vi "Workspace Experiment reload.vi"() -> ()   [LabVIEW 2023]
uses:
  <vilib>/Comparison/Equal/Equal Functor/Equal Functor.lvclass
  c59a542d-4e72-4e5b-a943-7cf77955b126.vi
  68731def-adea-4c2f-8935-8a66735695fa.vi
  <vilib>/Utility/sysdir.llb/System Directory Type.ctl
panel:
  out "output cluster":T1
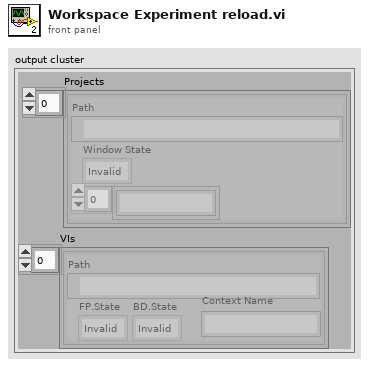
[diagram p1: front panel]
types:
  T1 = cluster{"Projects":cluster{"Path":path, "Window State":enum32{"Invalid", "Standard", "Closed", "Hidden", "Minimized", "Maximized"}, string[]}[], "VIs":cluster{"Path":path, "Context Name":string, "FP.State":enum32{"Invalid", "Standard", "Closed", "Hidden", "Minimized", "Maximized"}, "BD.State":enum32{"Invalid", "Standard", "Closed", "Hidden", "Minimized", "Maximized"}}[]}
  T2 = typedef "System Directory Type.ctl" = i32
  T3 = cluster{"Projects":cluster{"Path":path, "Window State":enum32{"Invalid", "Standard", "Closed", "Hidden", "Minimized", "Maximized"}, string[]}[], "VIs":cluster{"Path":path, string, "FP.State":enum32{"Invalid", "Standard", "Closed", "Hidden", "Minimized", "Maximized"}, "BD.State":enum32{"Invalid", "Standard", "Closed", "Hidden", "Minimized", "Maximized"}}[]}
  T4 = cluster{"Path":path, "Window State":enum32{"Invalid", "Standard", "Closed", "Hidden", "Minimized", "Maximized"}, string[]}[]
  T5 = cluster{"Path":path, string, "FP.State":enum32{"Invalid", "Standard", "Closed", "Hidden", "Minimized", "Maximized"}, "BD.State":enum32{"Invalid", "Standard", "Closed", "Hidden", "Minimized", "Maximized"}}[]
  T6 = enum32{"Invalid", "Standard", "Closed", "Hidden", "Minimized", "Maximized"}
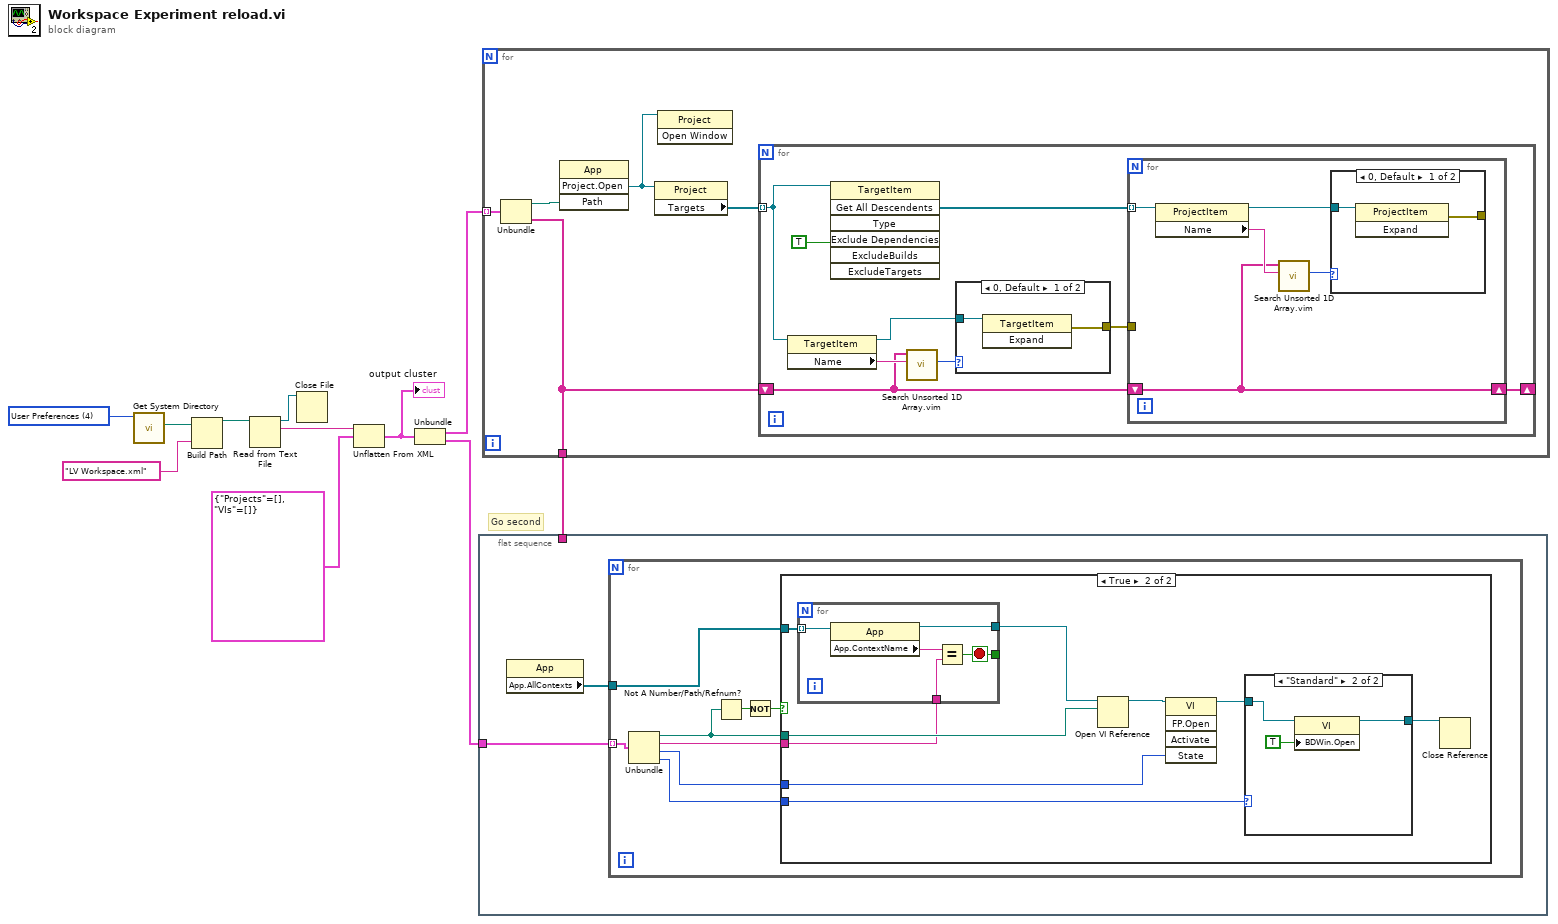
[diagram p0: block diagram]
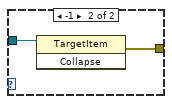
[diagram p4: hidden frame]
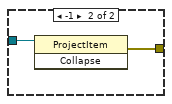
[diagram p5: hidden frame]
diagram:
  w3 = T2 4 items=["User Home"=0, "User Desktop"=1, "User Documents"=2, "User Application Data"=3, "User Preferences"=4, "User Temporary"=5, "Public Documents"=6, "Public Application Data"=7, "Public Preferences"=8, "Public Cache"=13, "System Core Libraries"=9, "System Installed Libraries"=10, "Application Files"=11, "Boot Volume Root"=12] ("system directory type")
  # "Go second"
  n1 = call <vilib>:"Get System Directory.vi"("system directory type"=w3) -> ("system directory"=w4:path)  [unwired: 10 in]
  n2 = Build Path(base path=w4, name or relative path="LV Workspace.xml") -> (appended path=w2:path)
  n3 = Read from Text File(file (use dialog)=w2) -> (refnum out=w6:refnum<file>, text=w7:string)  [unwired: 3 in, 2 out]
  n4 = Close File(refnum=w6) -> ()  [unwired: 1 in, 2 out]
  n5 = Unflatten From XML(xml string=w7, type=T3 {"Projects"=[], "VIs"=[]} ("output cluster")) -> (value=w8:T3)  [unwired: 1 in, 1 out]
  "output cluster" <- w8
  n6 = Unbundle(w8) -> ("Projects"=w10:T4, "VIs"=w11:T5)
  n7 = flat-sequence {
    tunnel: w11 -> [w13]
    tunnel: w1 -> [_]
    frame #0 {
      n8 = property class="App"() -> ("App.AllContexts"=w12:refnum<vi>[])  [unwired: 2 in, 2 out]
      n9 = for {
        tunnel: w13 -> [w21] mode=indexing
        tunnel: w12 -> [w17]
        n10 = Unbundle(w21) -> ("Path"=w18:path, w14:string, "FP.State"=w15:T6, "BD.State"=w16:T6)
        n11 = Not A Number/Path/Refnum?(number/path/refnum=w18) -> (NaN/Path/Refnum?=w20:bool)
        n12 = Not(x=w20) -> (.not. x?=w19:bool)
        n13 = case shown="True" w19 {
          tunnel: w18 -> [_ w30]
          tunnel: w15 -> [_ w28]
          tunnel: w16 -> [_ w27]
          tunnel: w17 -> [_ w24]
          tunnel: w14 -> [_ w23]
          frame False {
          }
          frame True {
            n14 = for {
              tunnel: w24 -> [w31] mode=indexing
              tunnel: w23 -> [w35]
              tunnel: [w32] -> w22
              tunnel: [w33] -> _
              stop <- w33 stop-if-true
              n15 = property class="App"(reference=w31) -> (reference out=w32:refnum<vi>, "App.ContextName"=w34:string)  [unwired: 1 in, 1 out]
              n16 = Equal?(x=w34, y=w35) -> (x = y?=w33:bool)
            }
            n17 = Open VI Reference(application reference (local)=w22, vi path=w30) -> (vi reference=w29:refnum<vi>)  [unwired: 4 in, 1 out]
            n18 = invoke class="VI" method="FP.Open"(reference=w29, "State"=w28) -> (reference out=w26:refnum<vi>)  [unwired: 3 in, 4 out]
            n19 = case shown="\"Standard\"" w27 {
              tunnel: w26 -> [w36 w39]
              tunnel: [w36 w37] -> w25
              frame "Invalid", Default {
              }
              frame "Standard" {
                n20 = property class="VI"(reference=w39, "BDWin.Open"=TRUE ("Block Diagram Window:Open")) -> (reference out=w37:refnum<vi>)  [unwired: 1 in, 1 out]
              }
            }
            n21 = Close Reference(reference=w25) -> ()  [unwired: 1 in, 1 out]
          }
        }
      }
    }
  }
  n22 = for {
    tunnel: w10 -> [w44] mode=indexing
    tunnel: [w41] -> w1
    n23 = Unbundle(w44) -> ("Path"=w43:path, w41:string[])  [unwired: 1 out]
    n24 = invoke class="App" method="Project.Open"("Path"=w43) -> ("Project:Open"=w40:refnum<vi>)  [unwired: 3 in, 3 out]
    n25 = property class="Project"(reference=w40) -> ("Targets"=w42:refnum<vi>[])  [unwired: 1 in, 2 out]
    n26 = invoke class="Project" method="Open Window"(reference=w40) -> ()  [unwired: 2 in, 3 out]
    n27 = for {
      tunnel: w42 -> [w51] mode=indexing
      shift-right: [w52] -> _
      shift-left: w41 -> [w48]
      n28 = property class="TargetItem"(reference=w51) -> (reference out=w46:refnum<vi>, "Name"=w49:string)  [unwired: 1 in, 1 out]
      n29 = invoke class="TargetItem" method="Get All Descendents"(reference=w51, "Exclude Dependencies"=TRUE ("ExcludeDependencies")) -> ("All Descendents"=w53:refnum<vi>[])  [unwired: 5 in, 6 out]
      n30 = call "Search Unsorted 1D Array.vim"("element"=w49, "unsorted 1D array"=w48) -> ("index of element"=w47:i32)  [unwired: 9 in]
      n31 = case shown="0, Default" w47 {
        tunnel: w46 -> [w55 w57]
        tunnel: [w54 w56] -> w45
        frame 0, Default {
          n32 = invoke class="TargetItem" method="Expand"(reference=w55) -> (error out=w54:errorcluster)  [unwired: 2 in, 2 out]
        }
        frame -1 {
          n33 = invoke class="TargetItem" method="Collapse"(reference=w57) -> (error out=w56:errorcluster)  [unwired: 2 in, 2 out]
        }
      }
      n34 = for {
        tunnel: w53 -> [w61] mode=indexing
        shift-right: [w58] -> w52
        shift-left: w48 -> [w58]
        tunnel: w45 -> [_]
        n35 = property class="ProjectItem"(reference=w61) -> (reference out=w62:refnum<vi>, "Name"=w60:string)  [unwired: 1 in, 1 out]
        n36 = call "Search Unsorted 1D Array.vim"("element"=w60, "unsorted 1D array"=w58) -> ("index of element"=w59:i32)  [unwired: 9 in]
        n37 = case shown="0, Default" w59 {
          tunnel: w62 -> [w64 w66]
          tunnel: [w63 w65] -> _
          frame 0, Default {
            n38 = invoke class="ProjectItem" method="Expand"(reference=w64) -> (error out=w63:errorcluster)  [unwired: 2 in, 2 out]
          }
          frame -1 {
            n39 = invoke class="ProjectItem" method="Collapse"(reference=w66) -> (error out=w65:errorcluster)  [unwired: 2 in, 2 out]
          }
        }
      }
    }
  }
